vi "Scripting_AlignToConnectorPane.vi"(8 "error in (no error)":errorcluster, 11 "VI Ref":refnum<vi>) -> (0 "error out":errorcluster)   [LabVIEW 2020, in "Scripting.lvclass"]
doc: "This VI arranges the Front Panel objects to match the Connector Pane layout"
uses:
  <resource>/Framework/Providers/Open_GDS/ClassProviders/Common/ScriptingFunctions/Scripting.lvclass
panel:
  # "Do not change the connector pane of this VI.\n\nSee the block diagram for directions on how to use this template."
  # "Specify the name of the Undo transaction"
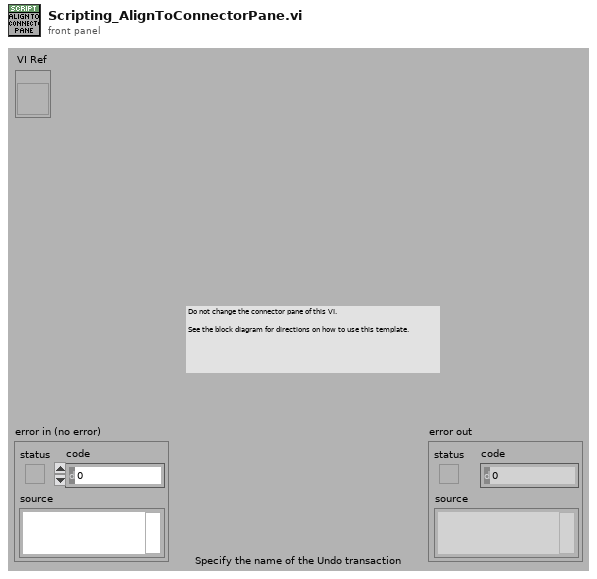
[diagram p1: front panel]
types:
  T1 = enum32{"Top Edges", "Vertical Centers", "Bottom Edges", "Left Edges", "Horizontal Centers", "Right Edges"}
  T2 = typedef "LVRectTypeDef.ctl" = cluster{"Left":i16, "Top":i16, "Right":i16, "Bottom":i16}
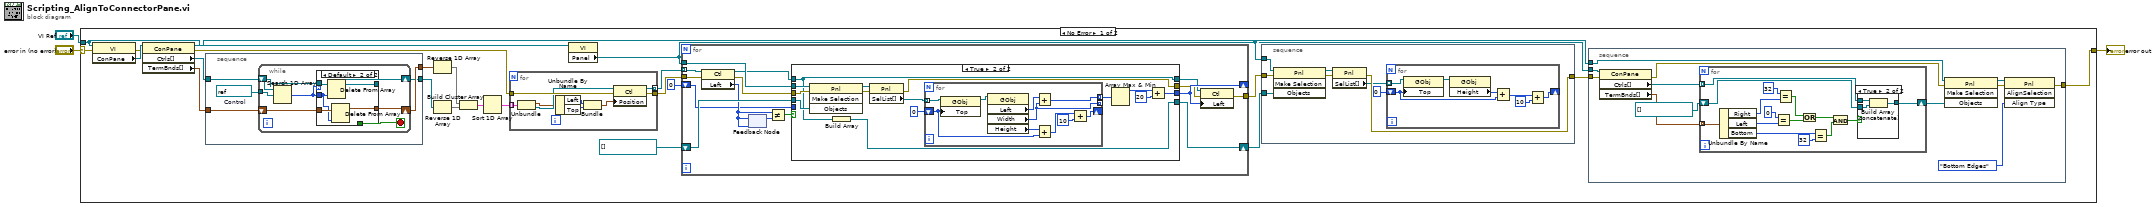
[diagram p0: block diagram]
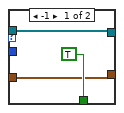
[diagram p3: hidden frame]
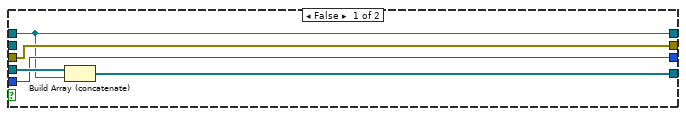
[diagram p4: hidden frame]
diagram:
  n1 = case shown="No Error" "error in (no error)" {
    selector: "error in (no error)" -> [w26 w146]
    tunnel: [w4 w146] -> w2
    tunnel: "VI Ref" -> [w25 _]
    frame No Error {
      n2 = property class="VI"(reference=w25, error in=w26) -> (error out=w13:errorcluster, "ConPane"=w19:refnum<vi>)  [unwired: 1 out]
      n3 = property class="ConPane"(reference=w19, error in=w13) -> (reference out=w14:refnum<vi>, error out=w10:errorcluster, "Ctrls[]"=w22:refnum<vi>[], "TermBnds[]"=w21:T2[])
      n4 = stacked-sequence {
        tunnel: [w77] -> w11
        tunnel: [w73] -> w12
        tunnel: w21 -> [w75]
        tunnel: w22 -> [w76]
        frame #0 {
          w74 = refnum<vi> refnum  # Control
          n5 = while {
            tunnel: w74 -> [w78]
            shift-right: [w83] -> w73
            shift-left: w76 -> [w84]
            shift-right: [w79] -> w77
            shift-left: w75 -> [w80]
            stop <- w81 stop-if-true
            n6 = Search 1D Array(1D array=w84, element=w78) -> (index of element=w82:i32)  [unwired: 1 in]
            n7 = case shown="Default" w82 {
              tunnel: w82 -> [_ w88]
              tunnel: w84 -> [w87 w92]
              tunnel: [w87 w91] -> w83
              tunnel: [TRUE _] -> w81
              tunnel: w80 -> [w85 w90]
              tunnel: [w85 w89] -> w79
              frame -1 {
              }
              frame Default {
                n8 = Delete From Array(array=w92, index=w88) -> (array with subset deleted=w91:refnum<vi>[])  [unwired: 1 in, 1 out]
                n9 = Delete From Array(array=w90, index=w88) -> (array with subset deleted=w89:T2[])  [unwired: 1 in, 1 out]
              }
            }
          }
        }
      }
      n10 = Reverse 1D Array(array=w11) -> (reversed array=w8:T2[])
      n11 = Reverse 1D Array(array=w12) -> (reversed array=w7:refnum<vi>[])
      n12 = Build Cluster Array(w8, w7) -> (w6:cluster{"Rectangle":T2, refnum<vi>}[])
      n13 = Sort 1D Array(array=w6) -> (sorted array=w5:cluster{"Rectangle":T2, refnum<vi>}[])
      n14 = for {
        tunnel: [w98] -> w23 mode=indexing
        tunnel: [w97] -> w15
        tunnel: w10 -> [w96]
        tunnel: w5 -> [w95] mode=indexing
        n15 = Unbundle(w95) -> ("Rectangle"=w93:T2, w94:refnum<vi>)
        n16 = Unbundle By Name(w93) -> ("Left"=w101:i16, "Top"=w100:i16)
        n17 = Bundle("Left"=w101, "Top"=w100) -> (w99:cluster{"Left":i16, "Top":i16})  [unwired: 1 in]
        n18 = property class="Ctl"(reference=w94, error in=w96, "Position"=w99) -> (reference out=w98:refnum<vi>, error out=w97:errorcluster)
      }
      n19 = property class="VI"(reference=w25) -> ("Panel"=w18:refnum<vi>)  [unwired: 1 in, 2 out]
      n20 = for {
        shift-right: [w115] -> w9
        shift-left: refnum<vi>[] [] -> [w114]
        shift-right: [w108] -> _
        shift-left: u32 0 ("Numeric") -> [w109]
        tunnel: w18 -> [w113]
        tunnel: w23 -> [w112] mode=indexing
        tunnel: [w106] -> w16
        tunnel: w15 -> [w104]
        n21 = property class="Ctl"(reference=w112, error in=w104) -> (reference out=w103:refnum<vi>, error out=w105:errorcluster, "Left"=w110:i32)
        n22 = feedback-in #1(w110) -> ()
        n23 = feedback #1(w110) -> (w116:i32)
        n24 = Not Equal?(x=w110, y=w116) -> (x != y?=w111:bool)
        n25 = case shown="True" w111 {
          tunnel: [w121 w135] -> w115
          tunnel: w114 -> [w120 w133]
          tunnel: [w119 w128] -> w108
          tunnel: w113 -> [_ w134]
          tunnel: w109 -> [w119 _]
          tunnel: [w118 w132] -> w107
          tunnel: w105 -> [w118 w131]
          tunnel: w103 -> [w117 w130]
          tunnel: [w117 w130] -> w102
          frame False {
            n26 = Build Array (concatenate)(w120, w117) -> (w121:refnum<vi>[])
          }
          frame True {
            n27 = invoke class="Pnl" method="Make Selection"(reference=w134, error in=w131, "Objects"=w133) -> (reference out=w126:refnum<vi>, error out=w125:errorcluster)  [unwired: 1 in, 2 out]
            n28 = Build Array(w130) -> (w135:refnum<vi>[])
            n29 = property class="Pnl"(reference=w126, error in=w125) -> (error out=w132:errorcluster, "SelList[]"=w123:refnum<vi>[])  [unwired: 1 out]
            n30 = for {
              tunnel: w123 -> [w138] mode=indexing
              tunnel: [w145] -> w122 mode=indexing
              tunnel: [w144] -> _ mode=indexing
              shift-right: [w139] -> _
              shift-left: u32 0 -> [w136]
              n31 = property class="GObj"(reference=w138, "Top"=w136) -> (reference out=w137:refnum<vi>)  [unwired: 1 in, 1 out]
              n32 = property class="GObj"(reference=w137) -> ("Left"=w143:i32, "Width"=w144:u32, "Height"=w142:u32)  [unwired: 1 in, 2 out]
              n33 = Add(x=w143, y=w144) -> (x+y=w145:u32)
              n34 = Add(x=w142, y=w136) -> (x+y=w141:u32)
              n35 = Add(x=w141, y=u32 10) -> (x+y=w139:u32)
            }
            n36 = Array Max & Min(array=w122) -> (max value=w129:u32)  [unwired: 3 out]
            n37 = Add(x=w129, y=u32 20) -> (x+y=w128:u32)
          }
        }
        n38 = property class="Ctl"(reference=w102, error in=w107, "Left"=w108) -> (error out=w106:errorcluster)  [unwired: 1 out]
      }
      n39 = stacked-sequence {
        tunnel: [w62] -> w17
        tunnel: w16 -> [w61]
        tunnel: w9 -> [w60]
        tunnel: w18 -> [w59]
        frame #0 {
          n40 = invoke class="Pnl" method="Make Selection"(reference=w59, error in=w61, "Objects"=w60) -> (reference out=w65:refnum<vi>, error out=w64:errorcluster)  [unwired: 1 in, 2 out]
          n41 = property class="Pnl"(reference=w65, error in=w64) -> (error out=w62:errorcluster, "SelList[]"=w58:refnum<vi>[])  [unwired: 1 out]
          n42 = for {
            tunnel: w58 -> [w68] mode=indexing
            shift-right: [w69] -> _
            shift-left: u32 0 -> [w66]
            n43 = property class="GObj"(reference=w68, "Top"=w66) -> (reference out=w67:refnum<vi>)  [unwired: 1 in, 1 out]
            n44 = property class="GObj"(reference=w67) -> ("Height"=w72:u32)  [unwired: 1 in, 2 out]
            n45 = Add(x=w72, y=w66) -> (x+y=w71:u32)
            n46 = Add(x=w71, y=u32 10) -> (x+y=w69:u32)
          }
        }
      }
      n47 = stacked-sequence {
        tunnel: [w27] -> w4
        tunnel: w17 -> [w30]
        tunnel: w14 -> [w28]
        tunnel: w18 -> [w35]
        frame #0 {
          n48 = property class="ConPane"(reference=w28, error in=w30) -> (error out=w29:errorcluster, "Ctrls[]"=w38:refnum<vi>[], "TermBnds[]"=w37:T2[])  [unwired: 1 out]
          n49 = for {
            tunnel: w38 -> [w42] mode=indexing
            tunnel: w37 -> [w53] mode=indexing
            shift-right: [w41] -> w34
            shift-left: refnum<vi>[] [] -> [w40]
            n50 = Unbundle By Name(w53) -> ("Right"=w48:i16, "Left"=w50:i16, "Bottom"=w52:i16)
            n51 = Equal?(x=i16 0, y=w50) -> (x = y?=w45:bool)
            n52 = Equal?(x=i16 32 ("right"), y=w48) -> (x = y?=w46:bool)
            n53 = Or(x=w46, y=w45) -> (x .or. y?=w44:bool)
            n54 = Equal?(x=w52, y=i16 32) -> (x = y?=w43:bool)
            n55 = And(x=w44, y=w43) -> (x .and. y?=w39:bool)
            n56 = case shown="True" w39 {
              tunnel: w42 -> [_ w57]
              tunnel: [w54 w56] -> w41
              tunnel: w40 -> [w54 w55]
              frame False {
              }
              frame True {
                n57 = Build Array (concatenate)(w57, w55) -> (w56:refnum<vi>[])
              }
            }
          }
          n58 = invoke class="Pnl" method="Make Selection"(reference=w35, error in=w29, "Objects"=w34) -> (reference out=w33:refnum<vi>, error out=w31:errorcluster)  [unwired: 1 in, 2 out]
          n59 = invoke class="Pnl" method="AlignSelection"(reference=w33, error in=w31, "Align Type"=T1."Bottom Edges") -> (error out=w27:errorcluster)  [unwired: 1 in, 3 out]
        }
      }
    }
    frame Error {
    }
  }
  "error out" <- w2
